vi "Teardown.vi"(11 "Event Transport in":refnum<class "Event Transport.lvclass">) -> (2 "Unheard Msgs":refnum<class "Msg.lvclass">[](array[class]))   [LabVIEW 2020, in "jettl.lvlib" / "Event Transport.lvlib" / "Event Transport.lvclass"]
uses:
  Event Transport.lvclass
  Msg/Msg.lvclass
  Event Transport.lvclass/Event Transport.ctl
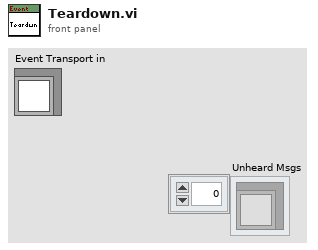
[diagram p1: front panel]
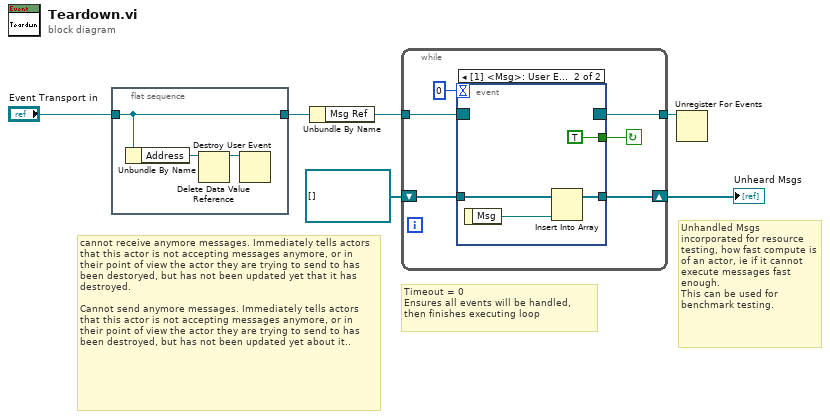
[diagram p0: block diagram]
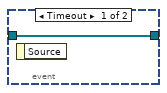
[diagram p2: hidden frame]
diagram:
  # "Unhandled Msgs incorporated for resource testing, how fast compute is of an actor, ie if it cannot execute messages fast enough.\nThis can be used for benchmark testing."
  # "Timeout = 0\nEnsures all events will be handled, then finishes executing loop"
  # "cannot receive anymore messages. Immediately tells actors that this actor is not accepting messages anymore, or in their point of view the actor they are trying to send to has been destoryed, but has not been updated yet that it has destroyed.\n\nCannot send anymore messages. Immediately tells actors that this actor is not accepting messages anymore, or in their point of view the actor they are trying to send to has been destroyed, but has not been updated yet about it.."
  n1 = flat-sequence {
    tunnel: "Event Transport in" -> [w9]
    tunnel: [w9] -> w2
    frame #0 {
      n2 = Unbundle By Name(w9) -> ("Address"=w7:refnum<data-value>)
      n3 = Delete Data Value Reference(data value reference=w7) -> (data value=w8:refnum<user-event>)  [unwired: 1 in, 1 out]
      n4 = Destroy User Event(user event=w8) -> ()  [unwired: 1 in, 1 out]
    }
  }
  n5 = Unbundle By Name(w2) -> ("Msg Ref"=w1:refnum<event-registration>)
  n6 = while {
    shift-right: [w14] -> w4
    shift-left: refnum<class "Msg.lvclass">[] [] -> [w15]
    tunnel: w1 -> [w13]
    tunnel: [w10] -> w5
    stop <- w12 continue-if-true
    n7 = event shown="[1] <Msg>: User Event" {
      selector: w13 -> [_ _]
      dyn-events: [_ _] -> w10
      timeout: 0 -> [_ _]
      tunnel: w15 -> [w16 w20]
      tunnel: [w16 w19] -> w14
      tunnel: [_ TRUE] -> w12
      event Timeout {
        n8 = event-data() -> ()  [unwired: 1 in, 1 out]
      }
      event User Event {
        n9 = event-data() -> ("Msg"=w18:refnum<class "Msg.lvclass">)  [unwired: 1 in]
        n10 = Insert Into Array(array=w20, new element=w18) -> (w19:refnum<class "Msg.lvclass">[])  [unwired: 1 in]
      }
    }
  }
  "Unheard Msgs" <- w4
  n11 = Unregister For Events(event registration refnum=w5) -> ()  [unwired: 1 in, 1 out]
